vi "Wfm Combine.vi"(8 "error in (no error)":errorcluster, 9 "Wfm3":waveform(dbl)={"t0"=timestamp(0 s since 1904-01-01), "dt"=1.0, "Y"=[100.0, 200.0, 300.0, 400.0, 500.0]}, 10 "Wfm2":waveform(dbl)={"t0"=timestamp(0 s since 1904-01-01), "dt"=1.0, "Y"=[10.0, 20.0, 30.0, 40.0]}, 11 "Wfm1":waveform(dbl)={"t0"=timestamp(0 s since 1904-01-01), "dt"=1.0, "Y"=[1.0, 2.0, 3.0]}) -> (0 "error out":errorcluster, 2 "Output Wfm":waveform(dbl)={"t0"=timestamp(0 s since 1904-01-01), "dt"=1.0, "Y"=[1.0, 2.0, 3.0, 10.0, 20.0, 30.0, 40.0, 100.0, 200.0, 300.0, 400.0, 500.0]})   [LabVIEW 2013]
doc: "Combines 3 waveforms into one using the dt from Wfm1."
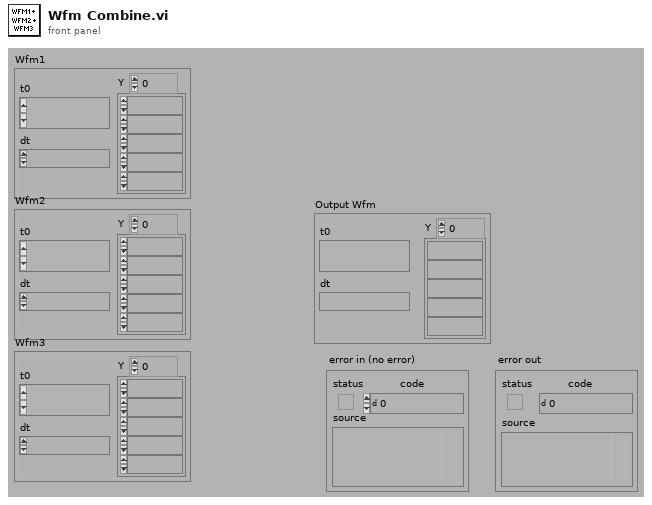
[diagram p1: front panel]
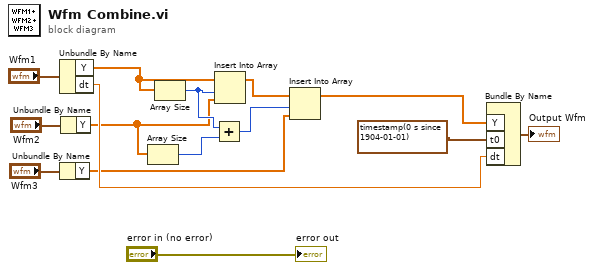
[diagram p0: block diagram]
diagram:
  n1 = Unbundle By Name("Wfm1") -> ("Y"=w14:dbl[], "dt"=w8:dbl)
  n2 = Unbundle By Name("Wfm3") -> ("Y"=w3:dbl[])
  n3 = Unbundle By Name("Wfm2") -> ("Y"=w2:dbl[])
  n4 = Array Size(array=w2) -> (size(s)=w5:i32)
  n5 = Array Size(array=w14) -> (size(s)=w6:i32)
  n6 = Add(x=w6, y=w5) -> (x+y=w4:i32)
  n7 = Insert Into Array(array=w14, index=w6, new element=w2) -> (w12:dbl[])
  n8 = Insert Into Array(array=w12, index=w4, new element=w3) -> (w10:dbl[])
  n9 = Bundle By Name("Y"=w10, "t0"=timestamp(0 s since 1904-01-01), "dt"=w8) -> (→"Output Wfm":waveform(dbl))  [unwired: 1 in]
  "error out" <- "error in (no error)"
